vi "ParseNumber.vi"(8 "error in (no error)":errorcluster, 10 "Index In":i32, 11 "JSON String":string) -> (0 "error out":errorcluster, 2 "Index Out":i32, 3 "JSON Tree":variant)   [LabVIEW 2014, in "i3-json.lvlib"]
doc: "Use this template to build a VI to use as a subVI."
uses:
  i3-json.lvlib
  JSON Types/JSON Type.ctl
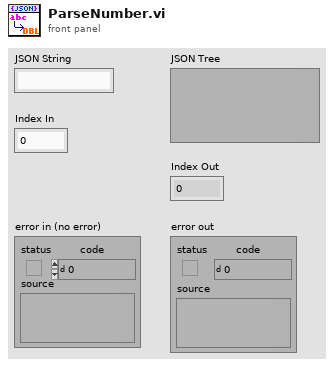
[diagram p1: front panel]
types:
  T1 = typedef "i3-json.lvlib/JSON Type.ctl" = enum8{"JSON Compatible", "JSON Array", "JSON Object", "JSON Null", "Double", "String", "Boolean", "Unknown"}
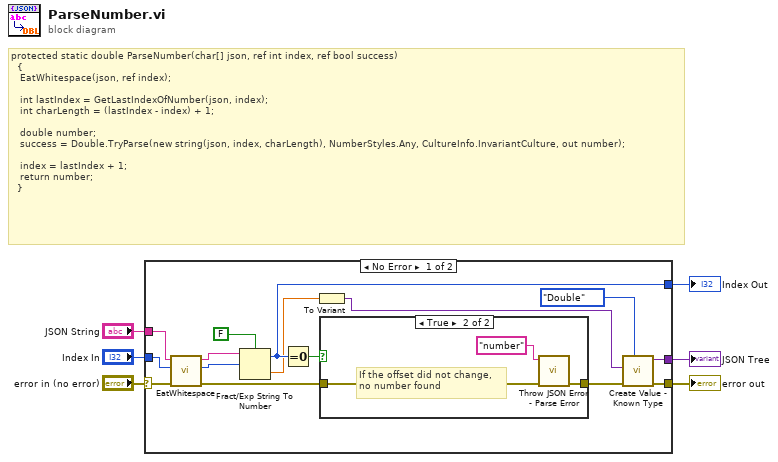
[diagram p0: block diagram]
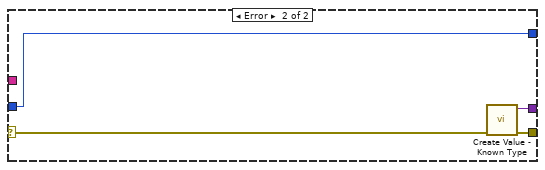
[diagram p3: hidden frame]
diagram:
  # "protected static double ParseNumber(char[] json, ref int index, ref bool success)\n\t\t{\n\t\t\tEatWhitespace(json, ref index);\n\n\t\t\tint lastIndex = GetLastIndexOfNumber(json, index);\n\t\t\tint charLength = (lastIndex - index) + 1;\n\n\t\t\tdouble number;\n\t\t\tsuccess = Double.TryParse(new string(json, index, charLength), NumberStyles.Any, CultureInfo.InvariantCulture, out number);\n\n\t\t\tindex = lastIndex + 1;\n\t\t\treturn number;\n\t\t}"
  n1 = case shown="No Error" "error in (no error)" {
    selector: "error in (no error)" -> [w20 w28]
    tunnel: [w16 w29] -> w5
    tunnel: [w15 w27] -> w4
    tunnel: "Index In" -> [w21 w26]
    tunnel: [w17 w26] -> w2
    tunnel: "JSON String" -> [w7 _]
    frame No Error {
      n2 = call "EatWhitespace.vi"("error in (no error)"=w20, "Index In"=w21, "JSON String"=w7) -> ("error out"=w10:errorcluster, "Index Out"=w18:i32, "JSON String Passthrough"=w19:string)  [unwired: 6 in]
      n3 = Fract/Exp String To Number(use system decimal point (T)=FALSE, string=w19, offset=w18) -> (offset past number=w17:i32, number=w12:dbl)  [unwired: 1 in]
      n4 = Equal To 0?(x=w17) -> (x = 0?=w11:bool)
      n5 = To Variant(anything=w12) -> (Variant=w13:variant)
      n6 = case shown="True" w11 {
        tunnel: w10 -> [w22 w24]
        tunnel: [w22 w23] -> w9
        frame False {
        }
        frame True {
          # "If the offset did not change,\nno number found"
          n7 = call "Throw JSON Error - Parse Error.vi"("error in (no error)"=w24, "datatype"="number") -> ("error out"=w23:errorcluster)  [unwired: 9 in]
        }
      }
      n8 = call "Create Value - Known Type.vi"("JSON Type"=JSON_Type."Double", "error in (no error)"=w9, "Value"=w13) -> ("error out"=w16:errorcluster, "JSON Tree"=w15:variant)  [unwired: 7 in]
    }
    frame Error {
      n9 = call "Create Value - Known Type.vi"("error in (no error)"=w28) -> ("error out"=w29:errorcluster, "JSON Tree"=w27:variant)  [unwired: 9 in]
    }
  }
  "error out" <- w5
  "Index Out" <- w2
  "JSON Tree" <- w4
